vi "TopLeft_Size_to_Rectangle.vi"(1 "Size":cluster{"width":i32, "height":i32}, 2 "Top Left":cluster{"left":i32, "top":i32}) -> (0 "Rectangle":T1)   [LabVIEW 2012]
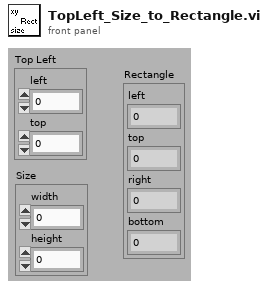
[diagram p1: front panel]
types:
  T1 = cluster{"left":i16, "top":i16, "right":i16, "bottom":i16}
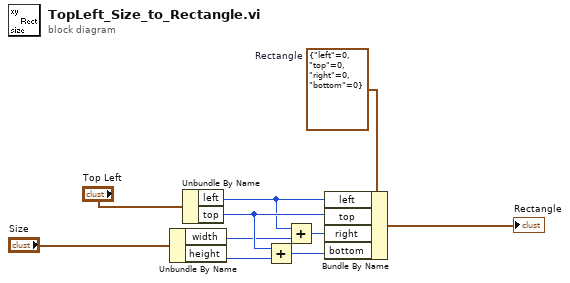
[diagram p0: block diagram]
diagram:
  w1 = T1 {"left"=0, "top"=0, "right"=0, "bottom"=0}  # Rectangle
  n1 = Unbundle By Name("Size") -> ("width"=w7:i32, "height"=w9:i32)
  n2 = Unbundle By Name("Top Left") -> ("left"=w6:i32, "top"=w10:i32)
  n3 = Add(x=w10, y=w9) -> (x+y=w8:i32)
  n4 = Add(x=w6, y=w7) -> (x+y=w5:i32)
  n5 = Bundle By Name(cluster=w1, "left"=w6, "top"=w10, "right"=w5, "bottom"=w8) -> (→"Rectangle":T1)
